vi "VI Tree.vi"   [LabVIEW 2020]
uses:
  d905f050-e613-4b45-93ad-a1a773cd948c.vi
  a5c1777a-5ee9-49d5-b883-b08c1e0241f4.vi
  c7e1df1c-7763-443f-8525-04ecc26e2465.vi
  G-Unicode.lvlib
  4abea8b1-338d-4d80-87cd-f7f18cc37e6a.vi
  138a86b6-19d0-4473-b672-eeb02bb9690a.vi
  82f20e20-a18c-4953-91e7-ac495547fece.vi
  5ed275a5-46b2-4734-aa74-f86eb5266c9a.vi
  c494f4e2-a60d-40c4-b576-910b447e17da.vi
  f086dd48-7e28-4fd3-bbdd-4644f1d55ea7.vi
  788fa793-ae5d-41ae-a63a-c7ce6a4c85e9.vi
  dd745465-5537-470d-ae7b-115044598478.vi
  c8bafa10-e4ca-402d-9a72-165dffe21227.vi
  66ecd2ef-1359-4cbe-bcdc-392ef8c6ce41.vi
  f0c140e7-13d8-46d3-8915-0b737f96c343.vi
  747e6b62-730e-4712-961a-61134bf14bd0.vi
  6ffdfe4f-ab24-45a8-ae48-fcad46a7d7c9.vi
  92286b1c-db29-4b0b-8f3a-6dd39cf11c11.vi
  9ef9509e-f996-465e-aaf8-2d458328f6da.vi
  bba91928-874c-410e-a14e-987a54761abf.vi
  8382f0bf-3b11-46d1-82a5-f4d8fe9eded6.vi
  2e2b5c76-486a-4838-bb23-bbeb66d8c2e1.vi
  b2c5cf29-7157-4dc6-917b-c4e0741bfc40.vi
  a07539d4-6e4b-4d2b-9e60-7aaf0706c2b1.vi
  2752499c-3eae-410a-a43f-5278ecf6bf83.vi
  3b0b9638-2d46-45bd-9f41-d3cd1bf3acb2.vi
  eb503347-6196-420f-b811-95c411e49e5f.vi
  af1edabf-1cb0-41f3-8ae9-a4d419df5b30.vi
  b0bd7731-091d-4174-a7fe-19175b04cc34.vi
  dea7b403-9e6f-4260-8221-ffad8176a7ef.vi
  59f9f0e1-81e7-4a80-a907-7160c16b316b.vi
  ec16afa1-090a-45bb-b28d-2fb822ce8a02.vi
  df61ee41-176e-4d26-836c-ef32aad2cc01.vi
  8099fc10-3e0e-4b81-9506-54922a16f28a.vi
  9c5bf8db-aea1-4f8b-8ec1-f1a248a2cbdb.vi
  1769f3e5-0cbf-42ce-ad94-688772e9396f.vi
  cb02f1ba-d678-43c3-9046-75a44fdfdb9f.vi
  86ecd8d1-94ca-4c0d-9fec-9dc574203941.vi
  Types/UTF-8 Path/UTF-8 Path.lvclass
  Types/UTF-8 String/UTF-8 String.lvclass
  Dialog & User Interface/Polymorphic VIs/Read Control Text/Read String Value (UTF-8 String).vi
  Dialog & User Interface/Polymorphic VIs/Write Control Text/Write String Value (UTF-8 String).vi
  127de910-6d92-46e2-b83f-85ccd560797a.vi
  cf740abb-9fb6-4f74-a6fa-1607993e9e8c.vi
  7d378eb3-8ee4-4c3c-98a6-b2ed373485c4.vi
  2e961d09-bdb5-4785-a636-2f6e90363a1a.vi
  fb6ecd53-a1ab-42cf-b8a0-906390218959.vi
  ca09041c-b4a4-48ad-8b93-5c9b7b740a87.vi
  cd7b11aa-46db-46a6-9351-89b39d7f8056.vi
  e669442a-b751-4256-846f-71c4eb969d91.vi
  3f5ebdfe-6788-492c-b8d0-3c20c1ebc2e1.vi
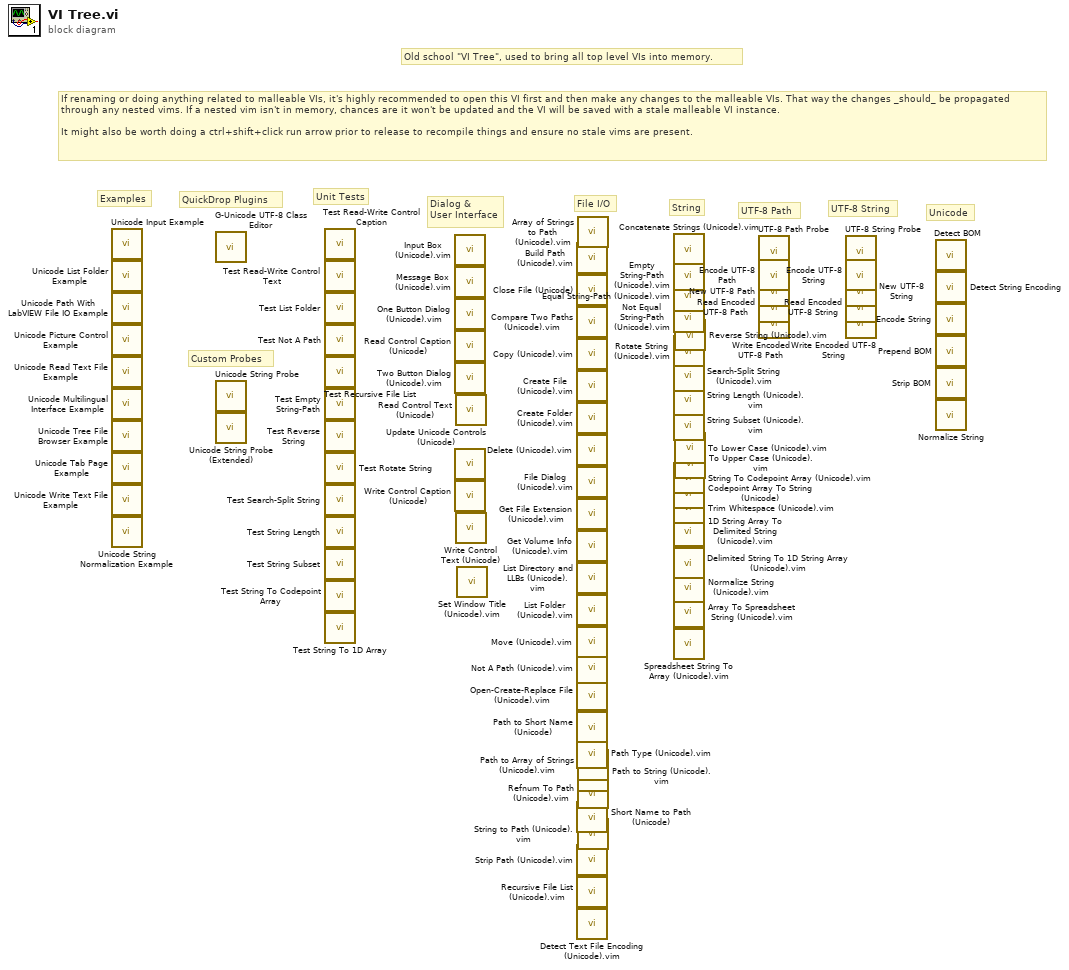
[diagram p0: block diagram]
diagram:
  # "Custom Probes"
  # "If renaming or doing anything related to malleable VIs, it's highly recommended to open this VI first and then make any changes to the malleable VIs. That way the changes _should_ be propagated through any nested vims. If a nested vim isn't in memory, chances are it won't be updated and the VI will be saved with a stale malleable VI instance.\n\nIt might also be worth doing a ctrl+shift+click run arrow prior to release to recompile things and ensure no stale vims are present."
  # "Old school \"VI Tree\", used to bring all top level VIs into memory."
  # "Unicode"
  # "UTF-8 String"
  # "UTF-8 Path"
  # "String"
  # "File I/O"
  # "Dialog &\nUser Interface"
  # "Unit Tests"
  # "QuickDrop Plugins"
  # "Examples"
  n1 = call "Unicode Input Example.vi"() -> ()  [unwired: 12 in]
  n2 = call "Unicode List Folder Example.vi"() -> ()  [unwired: 12 in]
  n3 = call "Unicode Path With LabVIEW File IO Example.vi"() -> ()  [unwired: 12 in]
  n4 = call "Unicode Picture Control Example.vi"() -> ()  [unwired: 12 in]
  n5 = call "Unicode Read Text File Example.vi"() -> ()  [unwired: 12 in]
  n6 = call "Unicode Multilingual Interface Example.vi"() -> ()  [unwired: 12 in]
  n7 = call "Unicode Tree File Browser Example.vi"() -> ()  [unwired: 12 in]
  n8 = call "Unicode Tab Page Example.vi"() -> ()  [unwired: 12 in]
  n9 = call "Unicode Write Text File Example.vi"() -> ()  [unwired: 12 in]
  n10 = call "Unicode String Normalization Example.vi"() -> ()  [unwired: 12 in]
  n11 = call "G-Unicode UTF-8 Class Editor.vi"() -> ()  [unwired: 10 in, 2 out]
  n12 = call "Unicode String Probe.vi"() -> ()  [unwired: 10 in, 2 out]
  n13 = call "Unicode String Probe (Extended).vi"() -> ()  [unwired: 10 in, 2 out]
  n14 = call "Test Read-Write Control Caption.vi"() -> ()  [unwired: 10 in, 2 out]
  n15 = call "Test Read-Write Control Text.vi"() -> ()  [unwired: 10 in, 2 out]
  n16 = call "Test List Folder.vi"() -> ()  [unwired: 10 in, 2 out]
  n17 = call "Test Not A Path.vi"() -> ()  [unwired: 10 in, 2 out]
  n18 = call "Test Recursive File List.vi"() -> ()  [unwired: 10 in, 2 out]
  n19 = call "Test Empty String-Path.vi"() -> ()  [unwired: 10 in, 2 out]
  n20 = call "Test Reverse String.vi"() -> ()  [unwired: 10 in, 2 out]
  n21 = call "Test Rotate String.vi"() -> ()  [unwired: 10 in, 2 out]
  n22 = call "Test Search-Split String.vi"() -> ()  [unwired: 10 in, 2 out]
  n23 = call "Test String Length.vi"() -> ()  [unwired: 10 in, 2 out]
  n24 = call "Test String Subset.vi"() -> ()  [unwired: 10 in, 2 out]
  n25 = call "Test String To Codepoint Array.vi"() -> ()  [unwired: 10 in, 2 out]
  n26 = call "Test String To 1D Array.vi"() -> ()  [unwired: 10 in, 2 out]
  n27 = call "Input Box (Unicode).vim"() -> ()  [unwired: 9 in, 3 out]
  n28 = call "Message Box (Unicode).vim"() -> ()  [unwired: 10 in, 2 out]
  n29 = call "One Button Dialog (Unicode).vim"() -> ()  [unwired: 6 in, 2 out]
  n30 = call "Read Control Caption (Unicode).vi"() -> ()  [unwired: 10 in, 2 out]
  n31 = call "Two Button Dialog (Unicode).vim"() -> ()  [unwired: 6 in, 2 out]
  n32 = call "Update Unicode Controls (Unicode).vi"() -> ()  [unwired: 9 in, 3 out]
  n33 = call "Write Control Caption (Unicode).vi"() -> ()  [unwired: 11 in, 1 out]
  n34 = call-poly "Read Control Text (Unicode).vi"() -> ()  [unwired: 10 in, 2 out]
  n35 = call-poly "Write Control Text (Unicode).vi"() -> ()  [unwired: 11 in, 1 out]
  n36 = call "Set Window Title (Unicode).vim"() -> ()  [unwired: 12 in]
  n37 = call "Build Path (Unicode).vim"() -> ()  [unwired: 8 in, 2 out]
  n38 = call "Close File (Unicode).vi"() -> ()  [unwired: 10 in, 2 out]
  n39 = call "Compare Two Paths (Unicode).vim"() -> ()  [unwired: 8 in, 4 out]
  n40 = call "Copy (Unicode).vim"() -> ()  [unwired: 9 in, 3 out]
  n41 = call "Create File (Unicode).vim"() -> ()  [unwired: 10 in, 2 out]
  n42 = call "Create Folder (Unicode).vim"() -> ()  [unwired: 9 in, 3 out]
  n43 = call "Delete (Unicode).vim"() -> ()  [unwired: 9 in, 3 out]
  n44 = call "File Dialog (Unicode).vim"() -> ()  [unwired: 8 in, 4 out]
  n45 = call "Get File Extension (Unicode).vim"() -> ()  [unwired: 7 in, 5 out]
  n46 = call "Get Volume Info (Unicode).vim"() -> ()  [unwired: 6 in, 6 out]
  n47 = call "List Directory and LLBs (Unicode).vim"() -> ()  [unwired: 8 in, 4 out]
  n48 = call "List Folder (Unicode).vim"() -> ()  [unwired: 8 in, 4 out]
  n49 = call "Move (Unicode).vim"() -> ()  [unwired: 9 in, 3 out]
  n50 = call "Not A Path (Unicode).vim"() -> ()  [unwired: 1 in, 1 out]
  n51 = call "Open-Create-Replace File (Unicode).vim"() -> ()  [unwired: 9 in, 3 out]
  n52 = call "Path to Short Name (Unicode).vi"() -> ()  [unwired: 10 in, 2 out]
  n53 = call "Path Type (Unicode).vim"() -> ()  [unwired: 1 in, 1 out]
  n54 = call "Short Name to Path (Unicode).vi"() -> ()  [unwired: 10 in, 2 out]
  n55 = call "Strip Path (Unicode).vim"() -> ()  [unwired: 7 in, 3 out]
  n56 = call "Recursive File List (Unicode).vim"() -> ()  [unwired: 7 in, 5 out]
  n57 = call "Detect Text File Encoding (Unicode).vim"() -> ()  [unwired: 9 in, 3 out]
  n58 = call "Array of Strings to Path (Unicode).vim"() -> ()  [unwired: 9 in, 2 out]
  n59 = call "Path to Array of Strings (Unicode).vim"() -> ()  [unwired: 8 in, 3 out]
  n60 = call "Path to String (Unicode).vim"() -> ()  [unwired: 10 in, 2 out]
  n61 = call "Refnum To Path (Unicode).vim"() -> ()  [unwired: 10 in, 2 out]
  n62 = call "String to Path (Unicode).vim"() -> ()  [unwired: 10 in, 2 out]
  n63 = call "Concatenate Strings (Unicode).vim"() -> ()  [unwired: 9 in, 2 out]
  n64 = call "Empty String-Path (Unicode).vim"() -> ()  [unwired: 1 in, 1 out]
  n65 = call "Equal String-Path (Unicode).vim"() -> ()  [unwired: 9 in, 2 out]
  n66 = call "Not Equal String-Path (Unicode).vim"() -> ()  [unwired: 9 in, 2 out]
  n67 = call "Rotate String (Unicode).vim"() -> ()  [unwired: 10 in, 2 out]
  n68 = call "Search-Split String (Unicode).vim"() -> ()  [unwired: 9 in, 3 out]
  n69 = call "String Length (Unicode).vim"() -> ()  [unwired: 10 in, 2 out]
  n70 = call "String Subset (Unicode).vim"() -> ()  [unwired: 10 in, 2 out]
  n71 = call "String To Codepoint Array (Unicode).vim"() -> ()  [unwired: 10 in, 2 out]
  n72 = call "Codepoint Array To String (Unicode).vi"() -> ()  [unwired: 10 in, 2 out]
  n73 = call "Trim Whitespace (Unicode).vim"() -> ()  [unwired: 9 in, 2 out]
  n74 = call "1D String Array To Delimited String (Unicode).vim"() -> ()  [unwired: 10 in, 2 out]
  n75 = call "Delimited String To 1D String Array (Unicode).vim"() -> ()  [unwired: 10 in, 2 out]
  n76 = call "Normalize String (Unicode).vim"() -> ()  [unwired: 9 in, 2 out]
  n77 = call "Array To Spreadsheet String (Unicode).vim"() -> ()  [unwired: 10 in, 2 out]
  n78 = call "Spreadsheet String To Array (Unicode).vim"() -> ()  [unwired: 10 in, 2 out]
  n79 = call "Reverse String (Unicode).vim"() -> ()  [unwired: 10 in, 2 out]
  n80 = call "To Lower Case (Unicode).vim"() -> ()  [unwired: 10 in, 2 out]
  n81 = call "To Upper Case (Unicode).vim"() -> ()  [unwired: 10 in, 2 out]
  n82 = call "UTF-8 Path Probe.vi"() -> ()  [unwired: 10 in, 2 out]
  n83 = call "Encode UTF-8 Path.vi"() -> ()  [unwired: 10 in, 2 out]
  n84 = call "New UTF-8 Path.vi"() -> ()  [unwired: 10 in, 2 out]
  n85 = call "Read Encoded UTF-8 Path.vi"() -> ()  [unwired: 11 in, 1 out]
  n86 = call "Write Encoded UTF-8 Path.vi"() -> ()  [unwired: 11 in, 1 out]
  n87 = call "UTF-8 String Probe.vi"() -> ()  [unwired: 10 in, 2 out]
  n88 = call "Encode UTF-8 String.vi"() -> ()  [unwired: 10 in, 2 out]
  n89 = call "New UTF-8 String.vi"() -> ()  [unwired: 10 in, 2 out]
  n90 = call "Read Encoded UTF-8 String.vi"() -> ()  [unwired: 11 in, 1 out]
  n91 = call "Write Encoded UTF-8 String.vi"() -> ()  [unwired: 11 in, 1 out]
  n92 = call "Detect BOM.vi"() -> ()  [unwired: 10 in, 2 out]
  n93 = call "Detect String Encoding.vi"() -> ()  [unwired: 9 in, 3 out]
  n94 = call "Encode String.vi"() -> ()  [unwired: 10 in, 2 out]
  n95 = call "Prepend BOM.vi"() -> ()  [unwired: 10 in, 2 out]
  n96 = call "Strip BOM.vi"() -> ()  [unwired: 9 in, 3 out]
  n97 = call "Normalize String.vi"() -> ()  [unwired: 10 in, 2 out]
